vi "Add Rows (Variant).vi"(7 "image path":path, 8 "error in (no error)":errorcluster, 9 "Data":variant[][](array[variant]), 11 "DataTable in":refnum<class "DataTable.lvclass">) -> (0 "error out":errorcluster, 3 "DataTable out":refnum<class "DataTable.lvclass">)   [LabVIEW 2013, in "DataGrid.lvlib" / "DataTable.lvclass"]
doc: "This allows any number of rows to be added to the datatable. The data must match the columns defined for the grid."
uses:
  DataTable.lvclass
  DataTable.lvclass/DataTable.ctl
  System.Data
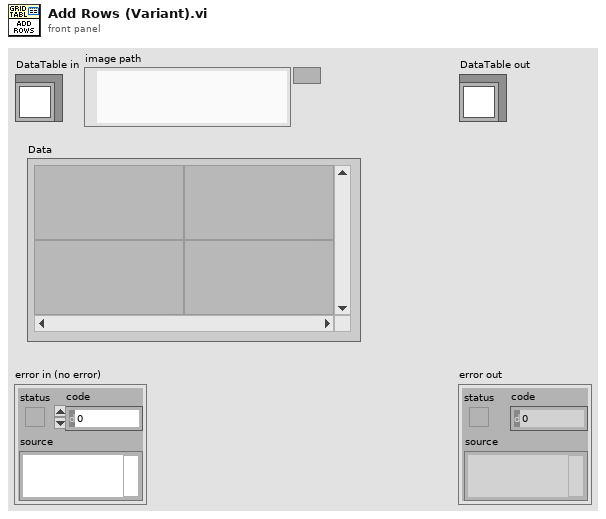
[diagram p1: front panel]
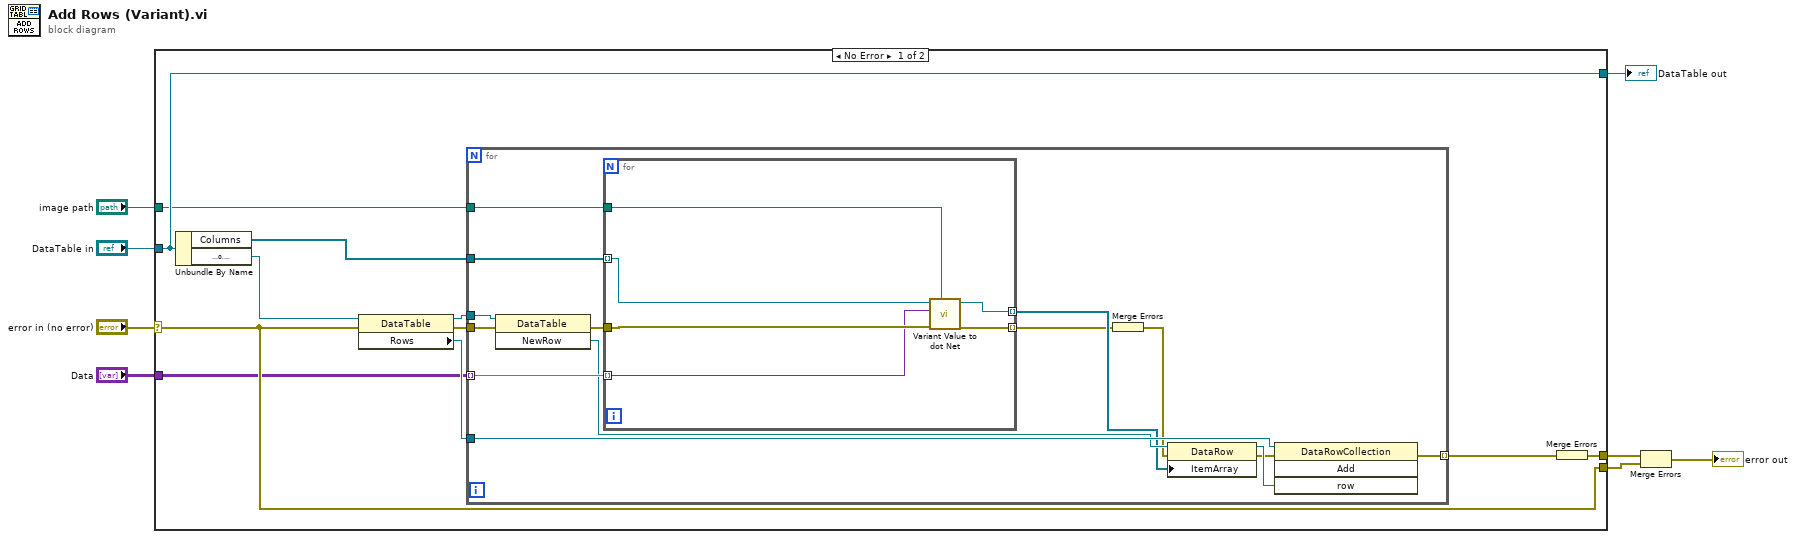
[diagram p0: block diagram]
diagram:
  n1 = case shown="No Error" "error in (no error)" {
    selector: "error in (no error)" -> [w15 w41]
    tunnel: [w15 w41] -> w7
    tunnel: [w16 w40] -> w5
    tunnel: "DataTable in" -> [w16 w40]
    tunnel: "Data" -> [w14 _]
    tunnel: [w12 _] -> w2
    tunnel: "image path" -> [w9 _]
    frame No Error {
      n2 = Unbundle By Name(w16) -> ("Columns"=w11:refnum<class "GridColumn.lvclass">[], "DataTable"=w10:refnum<k24>)
      n3 = property class="DataTable"(reference=w10, error in=w15) -> (reference out=w13:refnum<k24>, error out=w19:errorcluster, "Rows"=w18:refnum<k24>)
      n4 = for {
        tunnel: w18 -> [w32]
        tunnel: w13 -> [w33]
        tunnel: [w31] -> w17 mode=indexing
        tunnel: w14 -> [w30] mode=indexing
        tunnel: w19 -> [w22]
        tunnel: w11 -> [w21]
        tunnel: w9 -> [w20]
        n5 = invoke class="DataTable" method="NewRow"(reference=w33, error in=w22) -> (error out=w29:errorcluster, "NewRow"=w28:refnum<k24>)  [unwired: 1 in, 1 out]
        n6 = for {
          tunnel: w30 -> [w34] mode=indexing
          tunnel: [w39] -> w26 mode=indexing
          tunnel: w29 -> [w38]
          tunnel: [w37] -> w25 mode=indexing
          tunnel: w21 -> [w36] mode=indexing
          tunnel: w20 -> [w35]
          n7 = call "Variant Value to dot Net.vi"("image path"=w35, "error in (no error)"=w38, "element"=w34, "GridColumn in"=w36) -> ("error out"=w37:errorcluster, ".NET object"=w39:refnum<k24>)  [unwired: 6 in]
        }
        n8 = Merge Errors(w25) -> (w24:errorcluster)
        n9 = property class="DataRow"(reference=w28, error in=w24, "ItemArray"=w26) -> (reference out=w27:refnum<k24>, error out=w23:errorcluster)
        n10 = invoke class="DataRowCollection" method="Add"(reference=w32, error in=w23, "row"=w27) -> (error out=w31:errorcluster)  [unwired: 1 in, 3 out]
      }
      n11 = Merge Errors(w17) -> (w12:errorcluster)
    }
    frame Error {
    }
  }
  "DataTable out" <- w5
  n12 = Merge Errors(w2, w7) -> (→"error out":errorcluster)
